vi "Host_Manual_Control.vi"(8 "error in (no error)":errorcluster={"status"=FALSE, "code"=0, "source"="\"\""}, 10 "desired setpoint":string, 11 "Mode status":string) -> (0 "error out":errorcluster={"status"=FALSE, "code"=0, "source"="\"\""}, 2 "status ok":bool, 3 "CommandRequest":string)   [LabVIEW 2026]
doc: "INTENT: Request manual commands via Bridge. LOGIC: Require confirmed idle/manual state; submit typed command and show ACK/result."
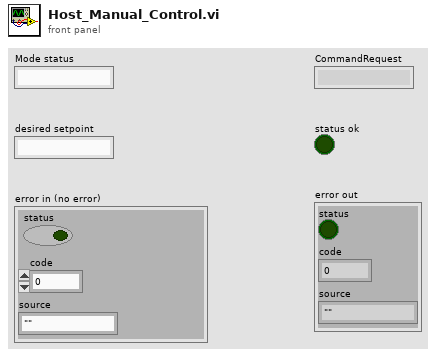
[diagram p1: front panel]
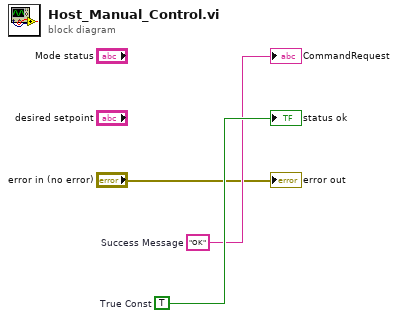
[diagram p0: block diagram]
diagram:
  w3 = TRUE  # True Const
  w2 = "OK"  # Success Message
  "CommandRequest" <- w2
  "status ok" <- w3
  "error out" <- "error in (no error)"
